vi "Code Conversion Paths.vi"(11 "error in":errorcluster) -> (2 "folders to ignore":path, 3 "deafult value setter vi":path, 4 "is project directory":path, 6 "io controls":path, 8 "get resource vi":path, 10 "error log path":path, 13 "deserializer":path, 14 "serializer":path, 15 "error out":errorcluster)   [LabVIEW 2021, in "Path Functions.lvlib"]
uses:
  Path Functions.lvlib
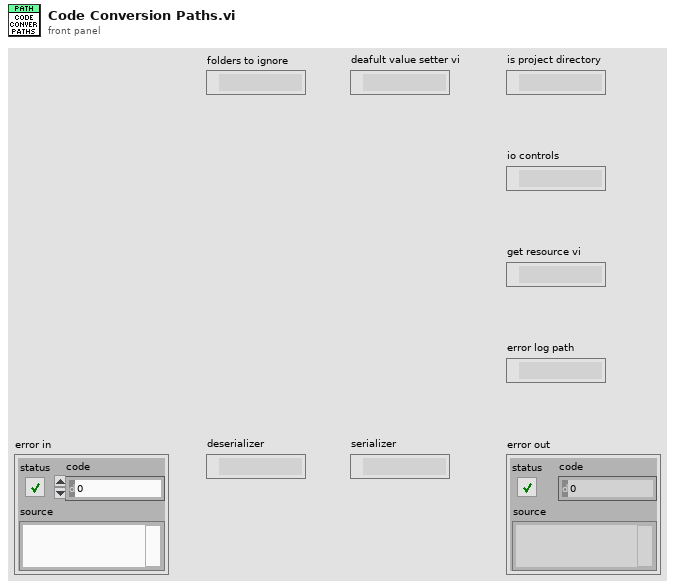
[diagram p1: front panel]
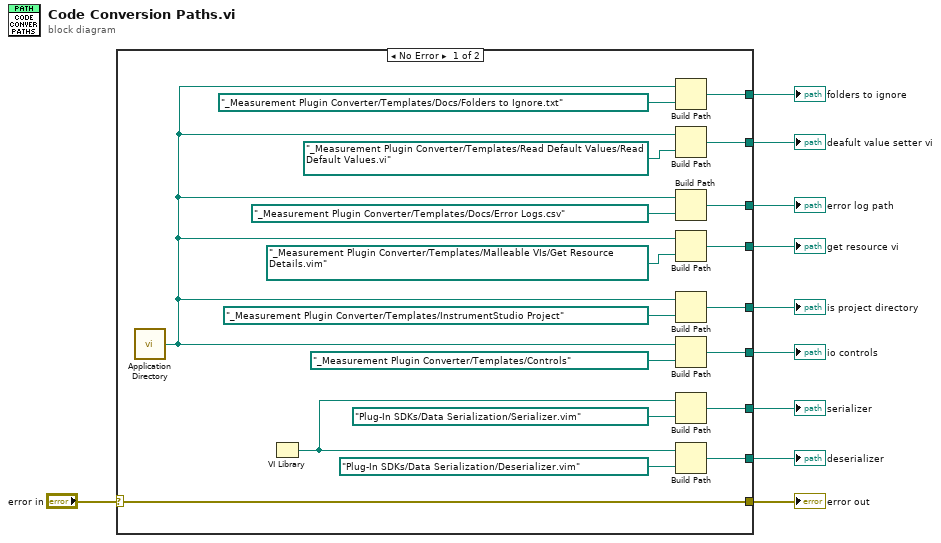
[diagram p0: block diagram]
diagram:
  n1 = case shown="No Error" "error in" {
    selector: "error in" -> [w25 w30]
    tunnel: [w29 _] -> w10
    tunnel: [w28 _] -> w9
    tunnel: [w27 _] -> w8
    tunnel: [w26 _] -> w7
    tunnel: [w25 w30] -> w6
    tunnel: [w24 _] -> w5
    tunnel: [w23 _] -> w4
    tunnel: [w18 _] -> w3
    tunnel: [w17 _] -> w2
    frame No Error {
      n2 = call <vilib>:"Application Directory.vi"() -> ("Application Directory"=w11:path)
      n3 = VI Library() -> (path=w16:path)
      n4 = Build Path(base path=w11, name or relative path=path "_Measurement Plugin Converter/Templates/Docs/Folders to Ignore.txt") -> (appended path=w23:path)
      n5 = Build Path(base path=w11, name or relative path=path "_Measurement Plugin Converter/Templates/Read Default Values/Read Default Values.vi") -> (appended path=w24:path)
      n6 = Build Path(base path=w11, name or relative path=path "_Measurement Plugin Converter/Templates/Docs/Error Logs.csv") -> (appended path=w26:path)
      n7 = Build Path(base path=w11, name or relative path=path "_Measurement Plugin Converter/Templates/Malleable VIs/Get Resource Details.vim") -> (appended path=w27:path)
      n8 = Build Path(base path=w11, name or relative path=path "_Measurement Plugin Converter/Templates/InstrumentStudio Project") -> (appended path=w29:path)
      n9 = Build Path(base path=w11, name or relative path=path "_Measurement Plugin Converter/Templates/Controls") -> (appended path=w28:path)
      n10 = Build Path(base path=w16, name or relative path=path "Plug-In SDKs/Data Serialization/Serializer.vim") -> (appended path=w17:path)
      n11 = Build Path(base path=w16, name or relative path=path "Plug-In SDKs/Data Serialization/Deserializer.vim") -> (appended path=w18:path)
    }
    frame Error {
    }
  }
  "error out" <- w6
  "is project directory" <- w10
  "io controls" <- w9
  "get resource vi" <- w8
  "error log path" <- w7
  "deserializer" <- w3
  "serializer" <- w2
  "deafult value setter vi" <- w5
  "folders to ignore" <- w4
